vi "New Logger.vi"(4 "dialog on failure? (T)":bool=TRUE, 5 "minimum log level (Info)":T1=enum."Info", 6 "enabled? (T)":bool=TRUE, 7 "name (\"Default\")":string="Default", 8 "error in (no error)":errorcluster, 9 "log handler (file handler)":refnum<class "Formatting Handler.lvclass">, 10 "log filter (none)":refnum<class "Filter.lvclass">, 11 "logger scope (all)":refnum<class "Scope.lvclass">) -> (0 "error out":errorcluster, 3 "logger":refnum<class "Logger.lvclass">)   [LabVIEW 2018, in "GLog.lvlib" / "Logger.lvclass"]
uses:
  Logger.lvclass
  extension/scope_interface/Scope.lvclass
  extension/formatting_handler_interface/Formatting Handler.lvclass
  extension/filter_interface/Filter.lvclass
  Log Levels.ctl
  Logger.lvclass/Logger.ctl
  configuration/handlers/file_handler/File Handler.lvclass
  C:/Users/Colin/Documents/software_projects/labview/glog/src/api/extension/formatting_handler_interface/Formatting Handler.lvclass
panel:
  # "Connector Pane"
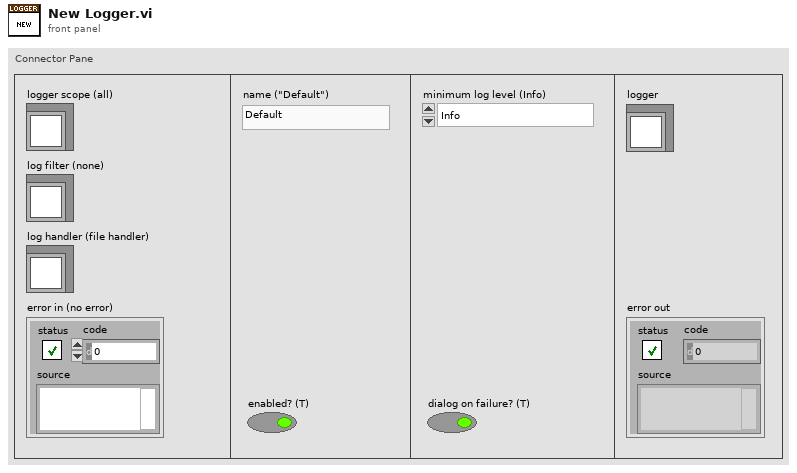
[diagram p1: front panel]
types:
  T1 = typedef "GLog.lvlib/Logger.lvclass/Log Levels.ctl" = enum16{"Trace", "Debug", "Info", "Warning", "Error", "Critical"}
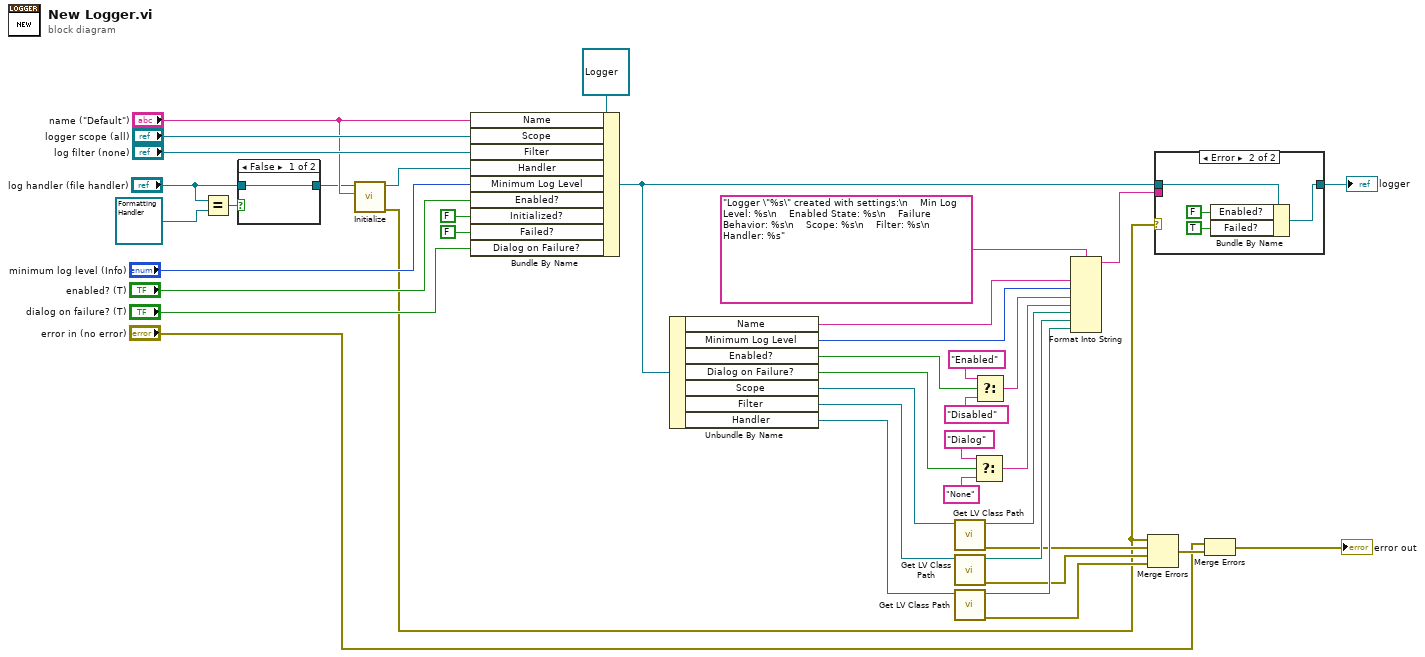
[diagram p0: block diagram]
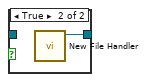
[diagram p2: hidden frame]
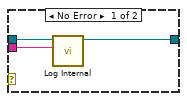
[diagram p3: hidden frame]
diagram:
  n1 = Equal?(x="log handler (file handler)", y=refnum<class "Formatting Handler.lvclass"> refnum ("log handler (file handler)")) -> (x = y?=w31:bool)
  n2 = case shown="False" w31 {
    tunnel: [w42 w43] -> w1
    tunnel: "log handler (file handler)" -> [w42 _]
    frame False {
    }
    frame True {
      n3 = call "New File Handler.vi"() -> ("file handler"=w43:refnum<class "File Handler.lvclass">)  [unwired: 9 in, 2 out]
    }
  }
  n4 = call-dynamic "Initialize.vi"("logger name"="name (\"Default\")", "handler in"=w1) -> ("error out"=w2:errorcluster, "handler out"=w37:refnum<class "Formatting Handler.lvclass">)  [unwired: 7 in, 1 out]
  n5 = Bundle By Name(cluster=refnum<class "Logger.lvclass"> refnum ("logger"), "Name"="name (\"Default\")", "Scope"="logger scope (all)", "Filter"="log filter (none)", "Handler"=w37, "Minimum Log Level"="minimum log level (Info)", "Enabled?"="enabled? (T)", "Initialized?"=FALSE ("Active?"), "Failed?"=FALSE, "Dialog on Failure?"="dialog on failure? (T)") -> (w29:refnum<class "Logger.lvclass">)
  n6 = Unbundle By Name(w29) -> ("Name"=w26:string, "Minimum Log Level"=w25:T1, "Enabled?"=w24:bool, "Dialog on Failure?"=w19:bool, "Scope"=w15:refnum<class "Scope.lvclass">, "Filter"=w14:refnum<class "Filter.lvclass">, "Handler"=w13:refnum<class "Formatting Handler.lvclass">)
  n7 = call <vilib>:"Get LV Class Path.vi"("object"=w15) -> ("error out"=w9:errorcluster, "class path"=w12:path)  [unwired: 9 in]
  n8 = call <vilib>:"Get LV Class Path.vi"("object"=w14) -> ("error out"=w8:errorcluster, "class path"=w11:path)  [unwired: 9 in]
  n9 = call <vilib>:"Get LV Class Path.vi"("object"=w13) -> ("error out"=w7:errorcluster, "class path"=w10:path)  [unwired: 9 in]
  n10 = Select(t="Dialog", s=w19, f="None") -> (s? t:f=w17:string)
  n11 = Select(t="Enabled", s=w24, f="Disabled") -> (s? t:f=w21:string)
  n12 = Format Into String(format string="Logger \"%s\" created with settings:\n    Min Log Level: %s\n    Enabled State: %s\n    Failure Behavior: %s\n    Scope: %s\n    Filter: %s\n    Handler: %s" ("message"), w26, w25, w21, w17, w12, w11, w10) -> (resulting string=w28:string)  [unwired: 2 in, 1 out]
  n13 = Merge Errors(w2, w9, w8, w7) -> (w6:errorcluster)
  n14 = case shown="Error" w2 {
    tunnel: w29 -> [w46 w50]
    tunnel: w28 -> [w45 _]
    tunnel: [w44 w49] -> w16
    frame No Error {
      n15 = call "Log Internal.vi"("message"=w45, "logger in"=w46) -> ("logger out"=w44:refnum<class "Logger.lvclass">)  [unwired: 9 in]
    }
    frame Error {
      n16 = Bundle By Name(cluster=w50, "Enabled?"=FALSE, "Failed?"=TRUE) -> (w49:refnum<class "Logger.lvclass">)
    }
  }
  "logger" <- w16
  n17 = Merge Errors("error in (no error)", w6) -> (→"error out":errorcluster)
